vi "DumpFileStart.vi"(6 "Overwrite":bool=TRUE, 9 "Data":dbl[][](array[numeric]), 10 "Path":path, 11 "DumpFileState":T1) -> (3 "DumpFileState out":T1)   [LabVIEW 2025]
uses:
  DumpFileState.ctl
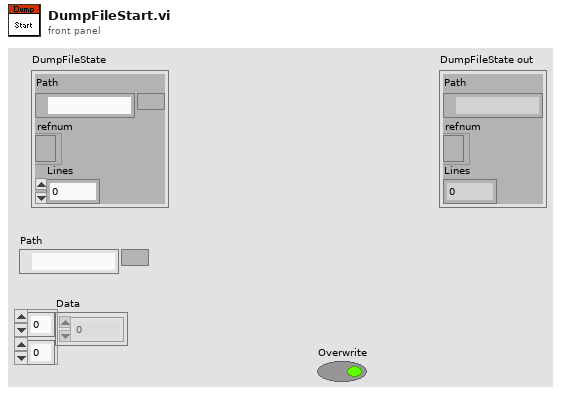
[diagram p1: front panel]
types:
  T1 = typedef "DumpFileState.ctl" = cluster{"Path":path, "refnum":refnum<file>, "Lines":i32}
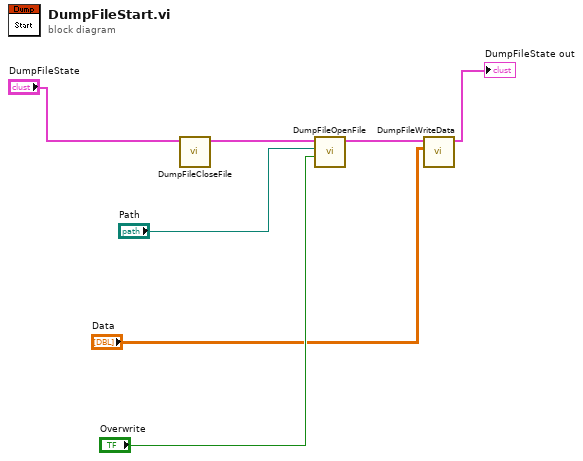
[diagram p0: block diagram]
diagram:
  n1 = call "DumpFileCloseFile.vi"("DumpFileState"="DumpFileState") -> ("DumpFileState out"=w6:T1)  [unwired: 10 in]
  n2 = call "DumpFileOpenFile.vi"("Overwrite"="Overwrite", "Path"="Path", "DumpFileState"=w6) -> ("DumpFileState out"=w3:T1)  [unwired: 8 in]
  n3 = call "DumpFileWriteData.vi"("Data"="Data", "DumpFileState"=w3) -> ("DumpFileState out"=→"DumpFileState out":T1)  [unwired: 9 in]
